vi "KYFG Open Ex.vi"(8 "error in (no error)":errorcluster, 9 "projectFile":string, 11 "index":i32) -> (0 "error out":errorcluster, 3 "handle":u32)   [LabVIEW 2023, in "KYFGLib_lv.lvlib"]
doc: "KYFG_API int KYFG_Scan(unsigned int *pids_info, int count); KYFG_API FGHANDLE KYFG_Open(int index);"
uses:
  KYFGLib_lv.lvlib
  KYFGLib.dll
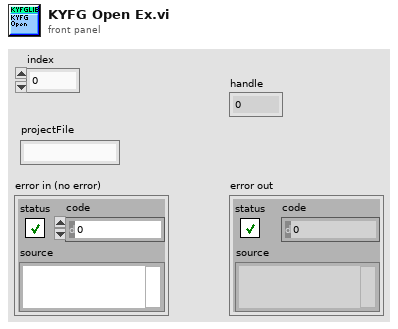
[diagram p1: front panel]
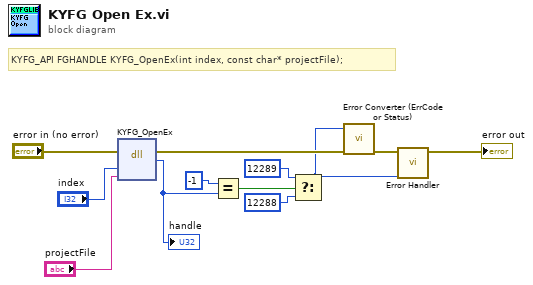
[diagram p0: block diagram]
diagram:
  # "KYFG_API FGHANDLE\tKYFG_OpenEx(int index, const char* projectFile);"
  n1 = dll-call lib="KYFGLib.dll" fn="KYFG_OpenEx"(error in="error in (no error)", "index"="index", "projectFile"="projectFile") -> (error out=w10:errorcluster, "return type"=w9:u32)  [unwired: 4 in, 1 out]
  "handle" <- w9
  n2 = Equal?(x=-1, y=w9) -> (x = y?=w8:bool)
  n3 = Select(t=12289, s=w8, f=12288) -> (s? t:f=w1:i32)
  n4 = call "Error Converter (ErrCode or Status).vi"("error in (no error)"=w10, "error code"=w1) -> ("error out"=w5:errorcluster)  [unwired: 9 in]
  n5 = call "Error Handler.vi"("Return Code"=w1, "Error In"=w5) -> ("Error Out"=→"error out":errorcluster)  [unwired: 9 in]
